vi "Stop Core.vi"(10 "final error code":i32, 11 "ZM-CM-communication_manager in":refnum<class "ZM-CM-communication_manager.lvclass">) -> (3 "ZM-CM-communication_manager out":refnum<class "ZM-CM-communication_manager.lvclass">)   [LabVIEW 2020, in "ZM-CM-communication_manager.lvlib" / "ZM-CM-communication_manager.lvclass"]
doc: "Stop Core override of the communication manager: Call Parent first, then ZM-CM-releaseProtocol closes the protocol. A release error is logged and passed on by releaseProtocol and ends here in Clear Errors, because AF's Stop Core has no error out."
uses:
  ZM-CM-communication_manager.lvclass
  <vilib>/ActorFramework/Actor/Actor.lvclass
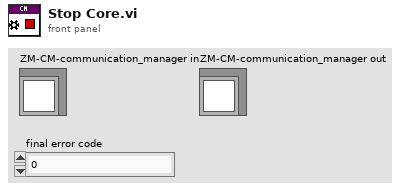
[diagram p1: front panel]
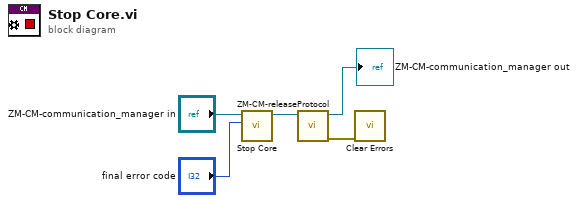
[diagram p0: block diagram]
diagram:
  n1 = call-parent "Stop Core.vi"("final error code"="final error code", "Actor in"="ZM-CM-communication_manager in") -> ("Actor out"=w2:refnum<class "ZM-CM-communication_manager.lvclass">)  [unwired: 9 in]
  n2 = call "ZM-CM-releaseProtocol.vi"("ZM-CM-communication_manager in"=w2) -> ("error out"=w1:errorcluster, "ZM-CM-communication_manager out"=→"ZM-CM-communication_manager out":refnum<class "ZM-CM-communication_manager.lvclass">)  [unwired: 9 in]
  n3 = call <vilib>:"Clear Errors.vi"("error in (no error)"=w1) -> ()  [unwired: 5 in, 2 out]
